vi "Barcode user prompt.vi"(8 "error in":errorcluster) -> (0 "error out":errorcluster, 2 "Time has Elapsed":bool, 3 "BARCODE":string)   [LabVIEW 2021]
uses:
  Control/Barcode.ctl
  Template/Main_VI/Control/Ini.ctl
panel:
  out "scan control":string caption="Input Barcode"
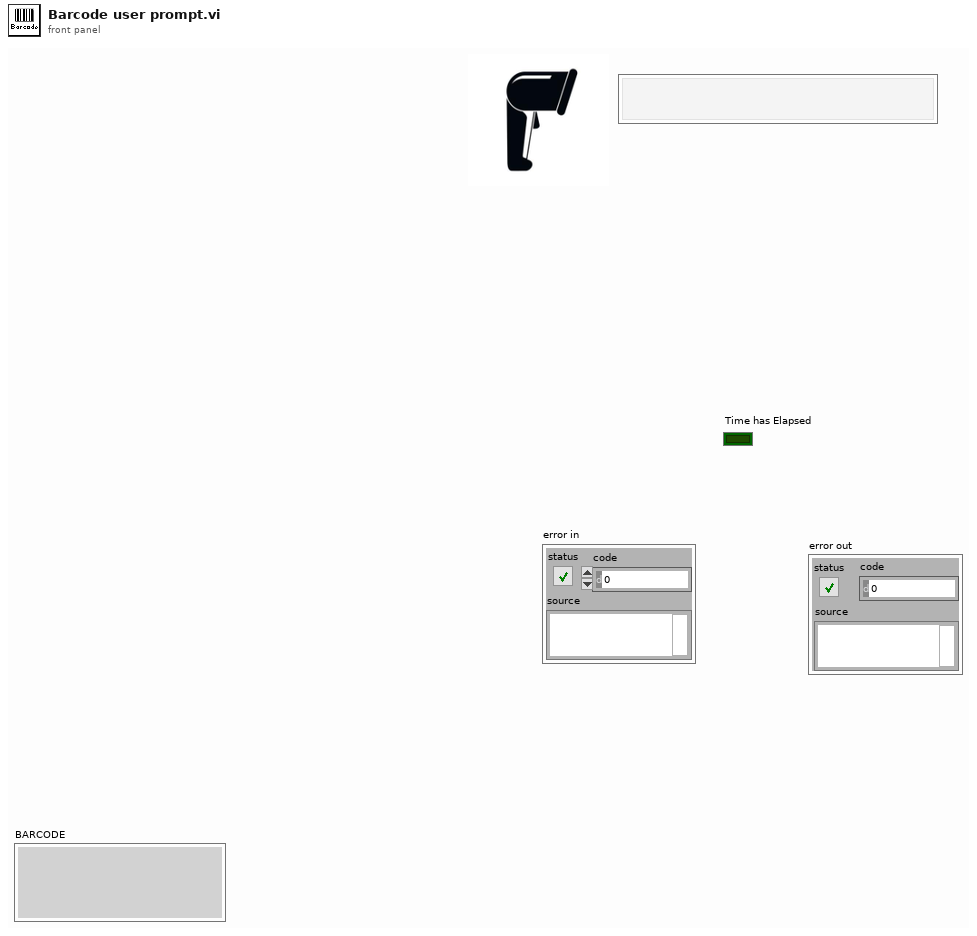
[diagram p1: front panel]
types:
  T1 = typedef "Barcode.ctl" = enum16{"Init", "Read", "Stop Reading", "Clear", "Close"}
  T2 = typedef "Ini.ctl" = enum16{"Write", "Read"}
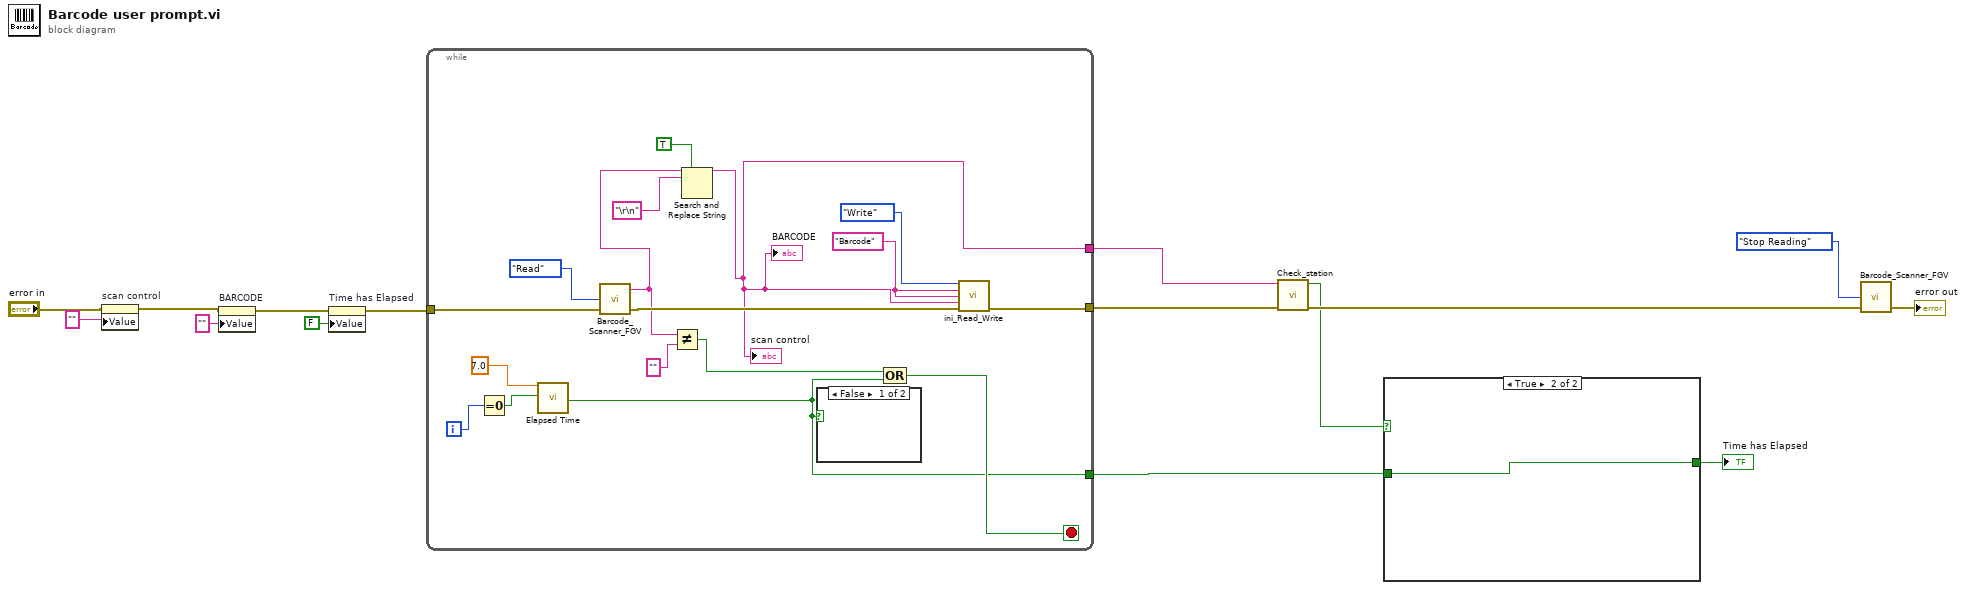
[diagram p0: block diagram]
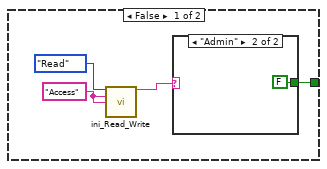
[diagram p2: hidden frame]
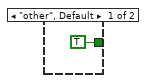
[diagram p3: hidden frame]
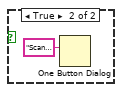
[diagram p4: hidden frame]
diagram:
  n1 = property on="scan control" class="Str"(error in="error in", "Value"="" ("scan control")) -> (error out=w13:errorcluster)  [unwired: 1 in, 1 out]
  n2 = property on="BARCODE" class="Str"(error in=w13, "Value"="" ("BARCODE")) -> (error out=w10:errorcluster)  [unwired: 1 in, 1 out]
  n3 = property on="Time has Elapsed" class="Bool (strict)"(error in=w10, "Value"=FALSE ("Time has Elapsed")) -> (error out=w9:errorcluster)  [unwired: 1 in, 1 out]
  n4 = while {
    tunnel: w9 -> [w23]
    tunnel: [w22] -> w6
    tunnel: [w20] -> w2
    tunnel: [w16] -> w1
    i -> [w31]
    stop <- w30 stop-if-true
    w25 = "Barcode" ("Write Section")
    n5 = Equal To 0?(x=w31) -> (x = 0?=w32:bool)
    n6 = call "Elapsed Time"("Time Target (s)"=7.0, "Reset"=w32) -> ("Time has Elapsed"=w20:bool)  [unwired: 10 in, 7 out]
    n7 = call "Barcode_Scanner_FGV.vi"("error in"=w23, "Action"=Barcode."Read") -> ("error out"=w24:errorcluster, "Barcode Data"=w17:string)  [unwired: 1 in, 1 out]
    n8 = Not Equal?(x=w17, y="") -> (x != y?=w28:bool)
    n9 = Search and Replace String(replace all?=TRUE ("replace all? (F)"), input string=w17, search string="\r\n") -> (result string=w16:string)  [unwired: 5 in, 3 out]
    "scan control" <- w16
    "BARCODE" <- w16
    n10 = case shown="False" w20 {
      frame False {
      }
      frame True {
        n11 = One Button Dialog(message="Scanning Failed Please Press Start Button") -> ()  [unwired: 1 in, 1 out]
      }
    }
    n12 = Compound Arithmetic op=OR(w28, w20) -> (w30:bool)
    n13 = call "ini_Read_Write.vi"(0:Ini."Write", "Write Section"=w25, "Write key"=w25, "Write"=w16, "error in (no error) 2"=w24) -> ("error in (no error) 3"=w22:errorcluster)  [unwired: 9 in, 1 out]
  }
  n14 = call "Check_station.vi"("error in"=w6, "Serial no"=w1) -> ("error out"=w5:errorcluster, "Result"=w4:bool)  [unwired: 8 in]
  n15 = case shown="True" w4 {
    tunnel: [w37 w40] -> w3
    tunnel: w2 -> [_ w40]
    frame False {
      w35 = "Access" ("Write")
      n16 = call "ini_Read_Write.vi"(0:Ini."Read", "Write Section"=w35, "Write key"=w35) -> ("value"=w34:string)  [unwired: 11 in, 1 out]
      n17 = case shown="\"Admin\"" w34 {
        tunnel: [TRUE ("Time has Elapsed") FALSE ("Time has Elapsed")] -> w37
        frame "other", Default {
        }
        frame "Admin" {
        }
      }
    }
    frame True {
    }
  }
  "Time has Elapsed" <- w3
  n18 = call "Barcode_Scanner_FGV.vi"("error in"=w5, "Action"=Barcode."Stop Reading") -> ("error out"=→"error out":errorcluster)  [unwired: 1 in, 2 out]
